vi "Test WebSockets Connection.vi"() -> ()   [LabVIEW 2013]
uses:
  <vilib>/LabVIEW Open Source Project/Connection/Connection/Connection.lvclass
  <vilib>/LabVIEW Open Source Project/MQTT Websockets Connection/MQTT_Websockets/Connection/WebsocketsConnection.lvclass
panel:
  out "ERROR 2":bool
  out "ERROR":bool
  out "server session error 2":errorcluster
  out "Bytes 2":u8[](array[numeric]) format="%08b"
  out "client session error 2":errorcluster
  out "value 2":dbl
  out "value":dbl
  out "listener error":errorcluster
  out "client session error":errorcluster
  out "server session error":errorcluster
  out "Bytes":u8[](array[numeric]) format="%08b"
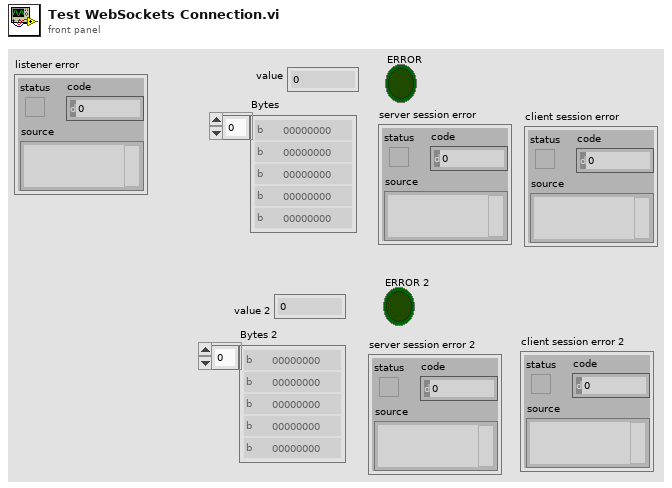
[diagram p1: front panel]
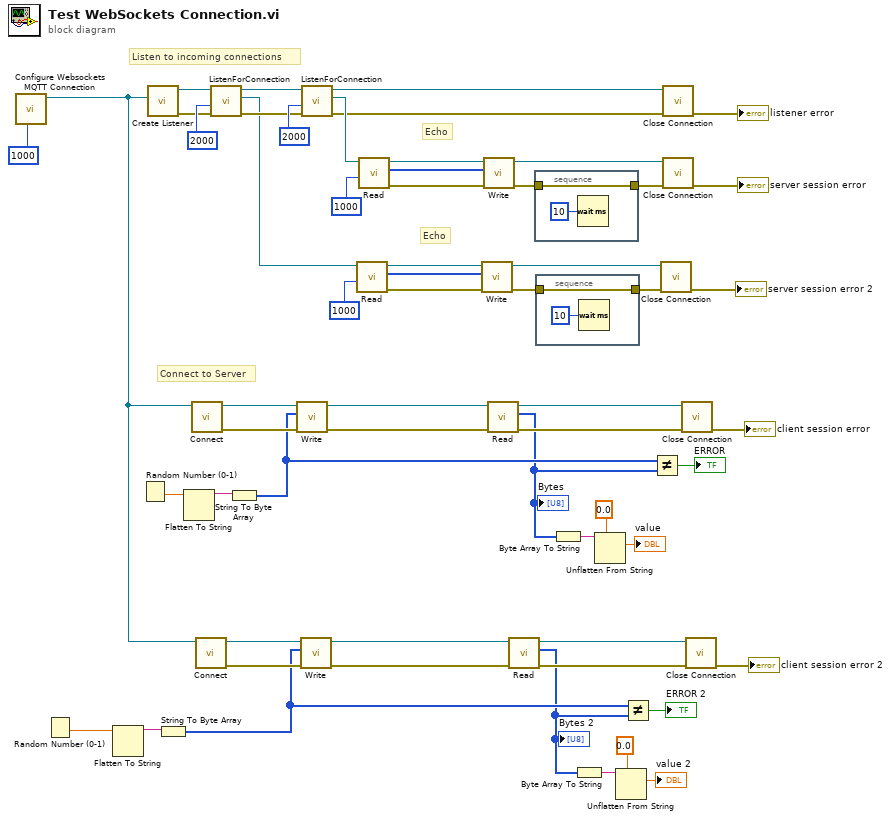
[diagram p0: block diagram]
diagram:
  # "Echo"
  # "Connect to Server"
  # "Echo"
  # "Listen to incoming connections"
  n1 = call <vilib>:"Configure Websockets MQTT Connection.vi"("timeout (5000 ms)"=1000 ("timeout (100ms)")) -> ("WSConnection"=w9:refnum<class "WebsocketsConnection.lvclass">)  [unwired: 9 in, 1 out]
  n2 = Random Number (0-1)() -> (number: 0 to 1=w30:dbl)
  n3 = Flatten To String(anything=w30) -> (data string=w31:string)  [unwired: 3 in, 2 out]
  n4 = Random Number (0-1)() -> (number: 0 to 1=w46:dbl)
  n5 = call <vilib>:"Create Listener.vi"("Connection Configuration"=w9) -> ("error out"=w1:errorcluster, "Listener"=w20:refnum<class "WebsocketsConnection.lvclass">)  [unwired: 9 in]
  n6 = String To Byte Array(string=w31) -> (unsigned byte array=w3:u8[])
  n7 = Flatten To String(anything=w46) -> (data string=w45:string)  [unwired: 3 in, 2 out]
  n8 = call <vilib>:"Connect.vi"("Connection in"=w9) -> ("error out"=w49:errorcluster, "Connection out"=w53:refnum<class "WebsocketsConnection.lvclass">)  [unwired: 9 in]
  n9 = call <vilib>:"Connect.vi"("Connection in"=w9) -> ("error out"=w29:errorcluster, "Connection out"=w26:refnum<class "WebsocketsConnection.lvclass">)  [unwired: 9 in]
  n10 = call <vilib>:"ListenForConnection.vi"("error in (no error)"=w1, "timeout (2000 ms)"=2000 ("bytes to read (100)"), "Listener"=w20) -> ("error out"=w18:errorcluster, "Connection"=w17:refnum<class "Connection.lvclass">, "Listener out"=w19:refnum<class "WebsocketsConnection.lvclass">)  [unwired: 5 in, 1 out]
  n11 = String To Byte Array(string=w45) -> (unsigned byte array=w7:u8[])
  n12 = call <vilib>:"Write.vi"("error in (no error)"=w49, "Bytes"=w7, "Connection in"=w53) -> ("error out"=w50:errorcluster, "Connection"=w52:refnum<class "WebsocketsConnection.lvclass">)  [unwired: 7 in]
  n13 = call <vilib>:"Write.vi"("error in (no error)"=w29, "Bytes"=w3, "Connection in"=w26) -> ("error out"=w28:errorcluster, "Connection"=w27:refnum<class "WebsocketsConnection.lvclass">)  [unwired: 7 in]
  n14 = call <vilib>:"ListenForConnection.vi"("error in (no error)"=w18, "timeout (2000 ms)"=2000 ("bytes to read (100)"), "Listener"=w19) -> ("error out"=w40:errorcluster, "Connection"=w56:refnum<class "Connection.lvclass">, "Listener out"=w58:refnum<class "WebsocketsConnection.lvclass">)  [unwired: 5 in, 1 out]
  n15 = call <vilib>:"Read.vi"("timeout (2000 ms)"=1000 ("bytes to read (100)"), "TCPConnection in"=w17) -> ("error out"=w25:errorcluster, "Bytes"=w24:u8[], "TCPConnection out"=w23:refnum<class "Connection.lvclass">)  [unwired: 5 in, 2 out]
  n16 = call <vilib>:"Read.vi"("timeout (2000 ms)"=1000 ("bytes to read (100)"), "TCPConnection in"=w56) -> ("error out"=w51:errorcluster, "Bytes"=w54:u8[], "TCPConnection out"=w55:refnum<class "Connection.lvclass">)  [unwired: 5 in, 2 out]
  n17 = call <vilib>:"Write.vi"("error in (no error)"=w25, "Bytes"=w24, "Connection in"=w23) -> ("error out"=w11:errorcluster, "Connection"=w14:refnum<class "Connection.lvclass">)  [unwired: 7 in]
  n18 = call <vilib>:"Write.vi"("error in (no error)"=w51, "Bytes"=w54, "Connection in"=w55) -> ("error out"=w13:errorcluster, "Connection"=w47:refnum<class "Connection.lvclass">)  [unwired: 7 in]
  n19 = call <vilib>:"Read.vi"("error in (no error)"=w50, "TCPConnection in"=w52) -> ("error out"=w15:errorcluster, "Bytes"=w6:u8[], "TCPConnection out"=w38:refnum<class "WebsocketsConnection.lvclass">)  [unwired: 5 in, 2 out]
  "Bytes" <- w6
  n20 = call <vilib>:"Read.vi"("error in (no error)"=w28, "TCPConnection in"=w27) -> ("error out"=w36:errorcluster, "Bytes"=w2:u8[], "TCPConnection out"=w37:refnum<class "WebsocketsConnection.lvclass">)  [unwired: 5 in, 2 out]
  "Bytes 2" <- w2
  n21 = stacked-sequence {
    tunnel: w13 -> [w60]
    tunnel: [w60] -> w12
    frame #0 {
      n22 = Wait (ms)(milliseconds to wait=u32 10) -> ()  [unwired: 1 out]
    }
  }
  n23 = stacked-sequence {
    tunnel: w11 -> [w62]
    tunnel: [w62] -> w10
    frame #0 {
      n24 = Wait (ms)(milliseconds to wait=u32 10) -> ()  [unwired: 1 out]
    }
  }
  n25 = Byte Array To String(unsigned byte array=w6) -> (string=w44:string)
  n26 = Byte Array To String(unsigned byte array=w2) -> (string=w32:string)
  n27 = Unflatten From String(type=0.0, binary string=w44) -> (value=→"value":dbl)  [unwired: 3 in, 2 out]
  n28 = Unflatten From String(type=0.0, binary string=w32) -> (value=→"value 2":dbl)  [unwired: 3 in, 2 out]
  n29 = Not Equal?(x=w3, y=w2) -> (x != y?=→"ERROR 2":bool)
  n30 = Not Equal?(x=w7, y=w6) -> (x != y?=→"ERROR":bool)
  n31 = call <vilib>:"Close Connection.vi"("error in (no error)"=w10, "Connection in"=w14) -> ("error out"=→"server session error 2":errorcluster)  [unwired: 8 in, 1 out]
  n32 = call <vilib>:"Close Connection.vi"("error in (no error)"=w40, "Connection in"=w58) -> ("error out"=→"listener error":errorcluster)  [unwired: 8 in, 1 out]
  n33 = call <vilib>:"Close Connection.vi"("error in (no error)"=w12, "Connection in"=w47) -> ("error out"=→"server session error":errorcluster)  [unwired: 8 in, 1 out]
  n34 = call <vilib>:"Close Connection.vi"("error in (no error)"=w15, "Connection in"=w38) -> ("error out"=→"client session error":errorcluster)  [unwired: 8 in, 1 out]
  n35 = call <vilib>:"Close Connection.vi"("error in (no error)"=w36, "Connection in"=w37) -> ("error out"=→"client session error 2":errorcluster)  [unwired: 8 in, 1 out]
